vi "Write Mouse Event Frame.vi"(11 "Replay Helper Loop In":T3) -> (3 "Replay Helper Loop Out":T3)   [LabVIEW 2026, in "Replay.lvlib"]
uses:
  Replay.lvlib
  User32.dll
  6371b789-ba5c-4556-852f-409c270b41c6.vi
  4cc629da-46f0-49b9-a83c-f938d5529bbf.vi
  modules/coordinator/src/Libraries/Core/global.vi
  modules/coordinator/src/Libraries/LUTVirtualKeySelector.ctl
  3d447ad9-a63f-4401-b3c5-38a1ebd2952b.vi
  <userlib>/_OpenG.lib/comparison/comparison.llb/openg_comparison__ogtk.lvlib
  6cc855f4-6c8e-465e-9ed0-3a173b85c1ed.vi
  <userlib>/_OpenG.lib/comparison/comparison.llb/U8 Changed__ogtk.vi
  modules/coordinator/src/Libraries/KeyboardLUTSelector.ctl
  Replay Helper Loop.ctl
  KeyboardReplayKey.ctl
panel:
  out "Key":T1(ring)
  out "Virtual Key":T2=164
  out "value out":errorcluster
  out "x = 0?":bool
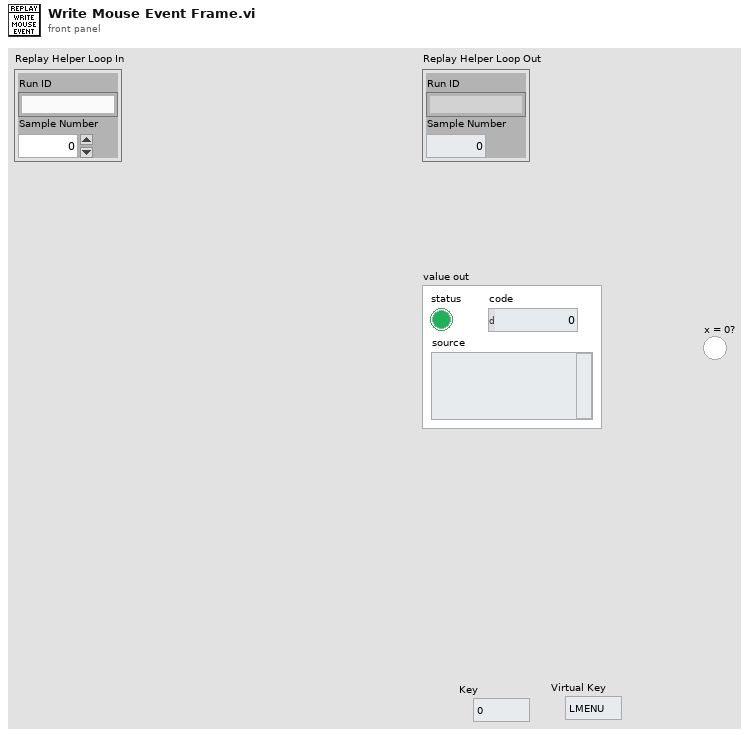
[diagram p1: front panel]
types:
  T1 = enum16{"0", "1", "2", "3", "4", "5", "6", "7", "8", "9", "A", "B", "C", "D", "E", "F", "G", "H", "I", "J", "K", "L", "M", "N", "O", "P", "Q", "R", "S", "T", "U", "V", "W", "X", "Y", "Z", "F1", "F2", "F3", "F4", "F5", "F6", "F7", "F8", "F9", "F10", "F11", "F12", "F13", "F14", "F15", "ADD", "BACK", "BACKSLASH", "CAPITAL", "COMMA", "DECIMAL", "DELETE", "DIVIDE", "DOWN", "END", "EQUALS", "ESCAPE", "GRAVE (`)", "HOME", "INSERT", "LBRACKET", "LCONTROL", "LEFT", "L ALT", "LSHIFT", "LWIN", "MINUS", "MULTIPLY", "NEXT", "NUMLOCK", "NUMPAD_0", "NUMPAD_1", "NUMPAD_2", "NUMPAD_3", "NUMPAD_4", "NUMPAD_5", "NUMPAD_6", "NUMPAD_7", "NUMPAD_8", "NUMPAD_9", "PAUSE", "PERIOD", "PRIOR (PG UP)", "RBRACKET", "RCONTROL", "RETURN", "RIGHT", "R ALT", "RSHIFT", "RWIN", "SCROLL", "SEMICOLON", "SLASH", "SPACE", "SUBTRACT", "TAB", "UP", "ENTER (num pad)", "' (quote)"}
  T2 = typedef "KeyboardReplayKey.ctl" = u8
  T3 = typedef "Replay.lvlib/Replay Helper Loop.ctl" = cluster{"Run ID":string, "Sample Number":i32}
  T4 = typedef "KeyboardLUTSelector.ctl" = enum16{"Initialize", "Get Keyboards Keys Pressed at Sample Number", "Assign Keyboard Key Press to Sample Number"}
  T5 = typedef "LUTVirtualKeySelector.ctl" = enum16{"Initialize", "Get Keyboard Event", "Set Keyboard Event"}
  T6 = typedef "KeyType.ctl" = enum16{"0", "1", "2", "3", "4", "5", "6", "7", "8", "9", "A", "B", "C", "D", "E", "F", "G", "H", "I", "J", "K", "L", "M", "N", "O", "P", "Q", "R", "S", "T", "U", "V", "W", "X", "Y", "Z", "F1", "F2", "F3", "F4", "F5", "F6", "F7", "F8", "F9", "F10", "F11", "F12", "F13", "F14", "F15", "ADD", "BACK", "BACKSLASH", "CAPITAL", "COMMA", "DECIMAL", "DELETE", "DIVIDE", "DOWN", "END", "EQUALS", "ESCAPE", "GRAVE (`)", "HOME", "INSERT", "LBRACKET", "LCONTROL", "LEFT", "L ALT", "LSHIFT", "LWIN", "MINUS", "MULTIPLY", "NEXT", "NUMLOCK", "NUMPAD_0", "NUMPAD_1", "NUMPAD_2", "NUMPAD_3", "NUMPAD_4", "NUMPAD_5", "NUMPAD_6", "NUMPAD_7", "NUMPAD_8", "NUMPAD_9", "PAUSE", "PERIOD", "PRIOR (PG UP)", "RBRACKET", "RCONTROL", "RETURN", "RIGHT", "R ALT", "RSHIFT", "RWIN", "SCROLL", "SEMICOLON", "SLASH", "SPACE", "SUBTRACT", "TAB", "UP", "ENTER (num pad)", "' (quote)"}
  T7 = cluster{"axis info":cluster{"Horizontal":i32, "Vertical":i32, "Scrolling":i32}, "button info":cluster{"button 1":bool, "button 2":bool, "button 3":bool, "button 4":bool}, "keyType":T6}
  T8 = cluster{"Horizontal":i32, "Vertical":i32, "Scrolling":i32}
  T9 = cluster{"button 1":bool, "button 2":bool, "button 3":bool, "button 4":bool}
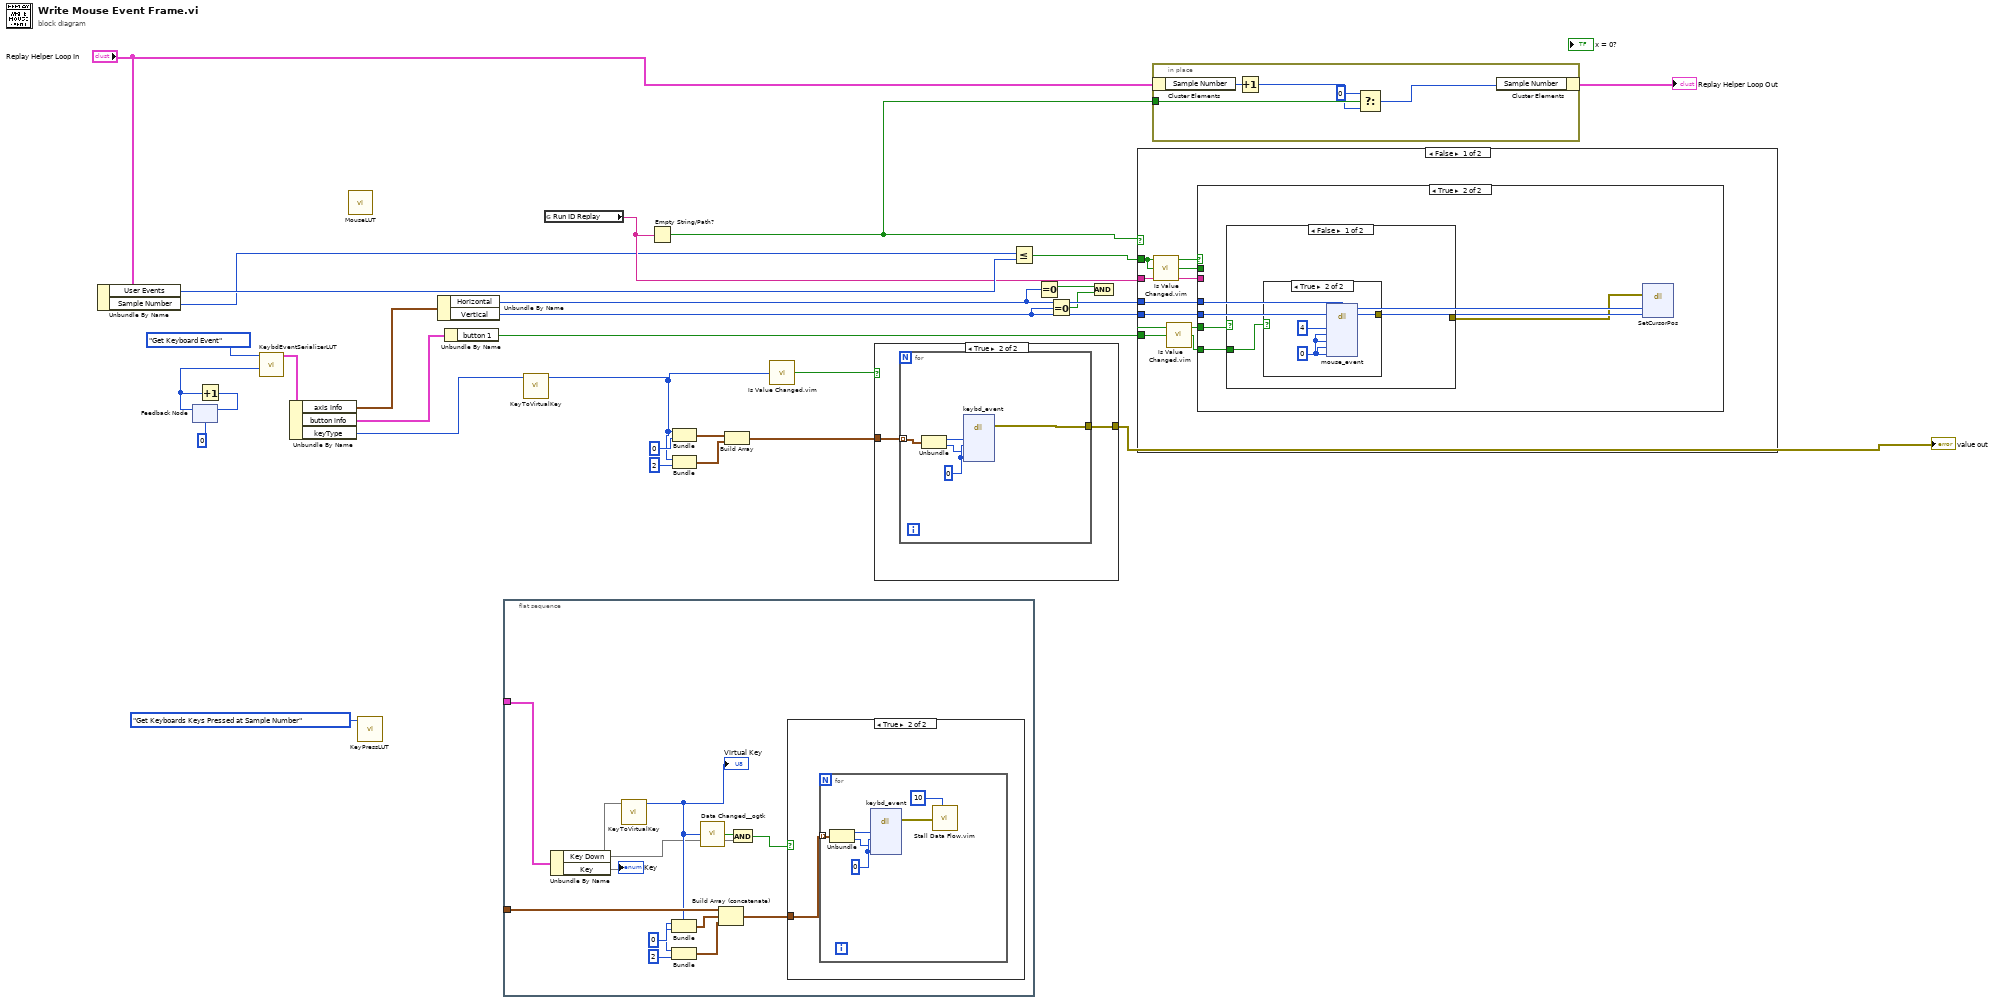
[diagram p0: block diagram]
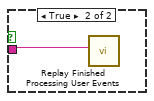
[diagram p5: hidden frame]
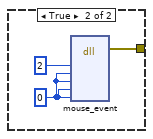
[diagram p8: hidden frame]
diagram:
  n1 = Unbundle By Name("Replay Helper Loop In") -> ("User Events"=w29:i32, "Sample Number"=w19:i32)
  n2 = feedback #1(u32 0 ("Iteration")) -> (w4:u32)
  n3 = Increment(x=w4) -> (x+1=w17:u32)
  n4 = feedback-in #1(w17) -> ()
  n5 = call "KeybdEventSerializerLUT.vi"("Iteration"=w4, "VirtualKeyLUTSelector"=LUTVirtualKeySelector."Get Keyboard Event") -> ("cluster"=w15:T7)  [unwired: 6 in, 3 out]
  n6 = Unbundle By Name(w15) -> ("axis info"=w14:T8, "button info"=w13:T9, "keyType"=w3:T6)
  n7 = call "MouseLUT.vi"() -> ()  [unwired: 9 in, 3 out]
  n8 = call "KeyPressLUT.vi"("LUT Selector"=KeyboardLUTSelector."Get Keyboards Keys Pressed at Sample Number") -> ()  [unwired: 9 in, 2 out]
  n9 = Unbundle By Name(w14) -> ("Horizontal"=w28:i32, "Vertical"=w27:i32)
  n10 = Unbundle By Name(w13) -> ("button 1"=w12:bool)
  n11 = flat-sequence {
    tunnel: _ -> [w41]
    tunnel: _ -> [w36]
    frame #0 {
      n12 = Unbundle By Name(w41) -> ("Key Down"=w31, "Key"=w40)
      "Key" <- w40
      n13 = call "KeyToVirtualKey.vi"("keyType Recorded"=w40) -> ("Virtual Key"=w33:T2)  [unwired: 9 in, 1 out]
      "Virtual Key" <- w33
      n14 = Bundle("Virtual Key"=w33, 0) -> (w38:cluster{"Virtual Key":T2, i32})  [unwired: 1 in]
      n15 = Bundle("Virtual Key"=w33, 2) -> (w39:cluster{"Virtual Key":T2, i32})  [unwired: 1 in]
      n16 = call-poly <userlib>:"Data Changed__ogtk.vi"("U8"=w33) -> ("Changed"=w32:bool)
      n17 = Build Array (concatenate)(w36, w38, w39) -> (w34:cluster{"Virtual Key":T2, i32}[])
      n18 = And(x=w32, y=w31) -> (x .and. y?=w30:bool)
      n19 = case shown="True" w30 {
        tunnel: w34 -> [_ w42]
        frame False {
        }
        frame True {
          n20 = for {
            tunnel: w42 -> [w47] mode=indexing
            w48 = u32 0 ("dwFlags")
            n21 = Unbundle(w47) -> ("Virtual Key"=w46:T2, w45:i32)
            n22 = dll-call lib="user32.dll" fn="keybd_event"("bVk"=w46, "bScan"=w48, "dwFlags"=w45, "dwExtraInfo"=w48) -> (error out=w44:errorcluster)  [unwired: 8 in, 1 out]
            n23 = call "Stall Data Flow.vim"("value in"=w44, "milliseconds to wait"=u32 10) -> ()  [unwired: 2 out]
          }
        }
      }
    }
  }
  n24 = call "KeyToVirtualKey.vi"("keyType Recorded"=w3) -> ("Virtual Key"=w6:T2)  [unwired: 9 in, 1 out]
  n25 = global read "global.vi" "Run ID Replay"() -> (w23:string)
  n26 = Empty String/Path?(string/path=w23) -> (empty?=w20:bool)
  n27 = Bundle("Virtual Key"=w6, 0) -> (w10:cluster{"Virtual Key":T2, i32})  [unwired: 1 in]
  n28 = Bundle("Virtual Key"=w6, 2) -> (w8:cluster{"Virtual Key":T2, i32})  [unwired: 1 in]
  n29 = Build Array(w10, w8) -> (w7:cluster{"Virtual Key":T2, i32}[])
  n30 = call "Is Value Changed.vim"("value"=w6) -> ("changed or first call?"=w5:bool)
  n31 = case shown="True" w5 {
    tunnel: w7 -> [_ w50]
    tunnel: [_ w49] -> w2
    frame False {
    }
    frame True {
      n32 = for {
        tunnel: w50 -> [w52] mode=indexing
        tunnel: [w51] -> w49
        w55 = u32 0 ("dwFlags")
        n33 = Unbundle(w52) -> ("Virtual Key"=w54:T2, w53:i32)
        n34 = dll-call lib="user32.dll" fn="keybd_event"("bVk"=w54, "bScan"=w55, "dwFlags"=w53, "dwExtraInfo"=w55) -> (error out=w51:errorcluster)  [unwired: 8 in, 1 out]
      }
    }
  }
  "value out" <- w2
  n35 = Less Or Equal?(x=w19, y=w29) -> (x <= y?=w24:bool)
  n36 = Equal To 0?(x=w28) -> (x = 0?=w26:bool)
  n37 = Equal To 0?(x=w27) -> (x = 0?=w25:bool)
  n38 = And(x=w26, y=w25) -> ()  [unwired: 1 out]
  n39 = case shown="False" w20 {
    tunnel: w12 -> [w62 _]
    tunnel: w23 -> [w60 _]
    tunnel: w24 -> [w59 _]
    tunnel: w28 -> [w57 _]
    tunnel: w27 -> [w56 _]
    frame False {
      n40 = call "Is Value Changed.vim"("value"=w59) -> ("changed or first call?"=w58:bool)
      n41 = call "Is Value Changed.vim"("value"=w62) -> ("changed or first call?"=w61:bool)
      n42 = case shown="True" w59 {
        tunnel: w57 -> [_ w70]
        tunnel: w56 -> [_ w69]
        tunnel: w62 -> [_ w68]
        tunnel: w61 -> [_ w67]
        tunnel: w60 -> [w63 _]
        tunnel: w58 -> [w64 _]
        frame False {
          # "Broadcast events finished here"
          n43 = case shown="False" w64 {
            tunnel: w63 -> [_ w65]
            frame False {
            }
            frame True {
              n44 = call "Replay Finished Processing User Events.vi"("Run ID"=w65) -> ()  [unwired: 10 in, 1 out]
            }
          }
        }
        frame True {
          n45 = case shown="False" w68 {
            tunnel: w67 -> [w72 w77]
            tunnel: [w71 w76] -> w66
            frame False {
              n46 = case shown="True" w72 {
                tunnel: [_ w73] -> w71
                frame False {
                }
                frame True {
                  w74 = u32 0 ("dy")
                  n47 = dll-call lib="user32.dll" fn="mouse_event"("dwFlags"=u32 4, "dx"=w74, "dy"=w74, "dwData"=w74, "dwExtraInfo"=w74) -> (error out=w73:errorcluster)  [unwired: 9 in, 1 out]
                }
              }
            }
            frame True {
              n48 = case shown="False" w77 {
                tunnel: [_ w78] -> w76
                frame False {
                }
                frame True {
                  w79 = u32 0 ("dy")
                  n49 = dll-call lib="user32.dll" fn="mouse_event"("dwFlags"=u32 2, "dx"=w79, "dy"=w79, "dwData"=w79, "dwExtraInfo"=w79) -> (error out=w78:errorcluster)  [unwired: 9 in, 1 out]
                }
              }
            }
          }
          n50 = dll-call lib="User32.dll" fn="SetCursorPos" label="SetCursorPos (User32.dll)"(error in=w66, w70, w69) -> ()  [unwired: 4 in, 3 out]
        }
      }
    }
    frame True {
    }
  }
  n51 = in-place {
    in-place-border: w20 -> [w85]
    n52 = in-place-cluster #2("Replay Helper Loop In") -> ("Sample Number"=w84:i32)
    n53 = Increment(x=w84) -> (x+1=w83:i32)
    n54 = Select(t=0, s=w85, f=w83) -> (s? t:f=w82:i32)
    n55 = in-place-cluster #2("Sample Number"=w82) -> (→"Replay Helper Loop Out":T3)
  }
